vi "Acquire Data.vi"(7 "user event":T2, 8 "error in (no error)":errorcluster, 9 "UI Refs":T1, 10 "Waveforms":waveform(dbl)[](array[waveform]), 11 "H1 Hydraulic":refnum<class "H1 Hydraulic.lvclass">) -> (0 "error out":errorcluster, 3 "H1 Hydraulic out":refnum<class "H1 Hydraulic.lvclass">)   [LabVIEW 2025, in "H1 Plotter.lvlib" / "H1 Hydraulic.lvclass"]
uses:
  H1 Hydraulic.lvclass
  Users/Public/Documents/Sandia National Labs/TSS Plugin/CEF.lvlibp/Node/UserEventRef.ctl
  Users/Public/Documents/Sandia National Labs/TSS Plugin/Tests/XY Plotter.lvlibp/XY Plotter configuration/Read XY Plotter.vi
  Users/Public/Documents/Sandia National Labs/TSS Plugin/CEF.lvlibp/serializable configuration/CEF_serializable configuration.lvclass
  H1 Hydraulic.lvclass/H1 Hydraulic.ctl
  Users/Public/Documents/Sandia National Labs/TSS Plugin/Tests/XY Plotter.lvlibp/XY  Plotter/XY Plotter.lvclass
  Users/Public/Documents/Sandia National Labs/TSS Plugin/CEF.lvlibp/Node/CEF_Node.lvclass
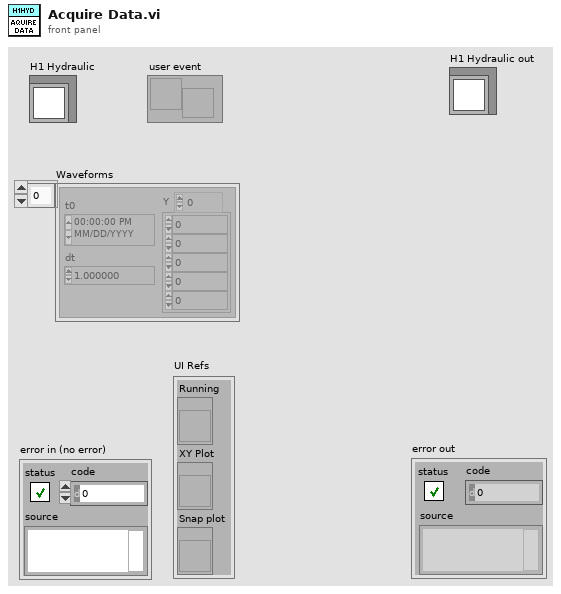
[diagram p1: front panel]
types:
  T1 = cluster{"Running":refnum<vi>, "XY Plot":refnum<vi>, "Snap plot":refnum<vi>}
  T2 = typedef "CEF.lvlibp/CEF_Node.lvclass/UserEventRef.ctl" = refnum<user-event>
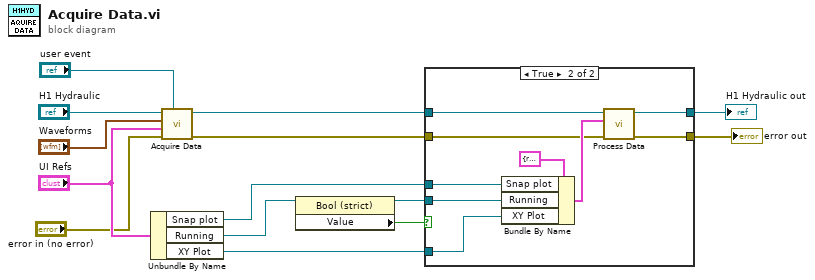
[diagram p0: block diagram]
diagram:
  n1 = Unbundle By Name("UI Refs") -> ("Snap plot"=w8:refnum<vi>, "Running"=w9:refnum<vi>, "XY Plot"=w10:refnum<vi>)
  n2 = call-parent "Acquire Data.vi"("user event"="user event", "error in (no error)"="error in (no error)", "UI Refs"="UI Refs", "Waveforms"="Waveforms", "XY Plotter"="H1 Hydraulic") -> ("error out"=w1:errorcluster, "XY Plotter out"=w6:refnum<class "H1 Hydraulic.lvclass">)  [unwired: 5 in]
  n3 = property class="Bool (strict)"(reference=w9) -> (reference out=w14:refnum<vi>, "Value"=w13:bool)  [unwired: 1 in, 1 out]
  n4 = case shown="True" w13 {
    tunnel: [w16 w25] -> w11
    tunnel: w14 -> [_ w24]
    tunnel: w6 -> [w16 w23]
    tunnel: [w15 w17] -> w12
    tunnel: w10 -> [_ w22]
    tunnel: w8 -> [_ w21]
    tunnel: w1 -> [w15 w18]
    frame False {
    }
    frame True {
      n5 = Bundle By Name(cluster=T1 {"Running"=refnum, "XY Plot"=refnum, "Snap plot"=refnum} ("UI Refs"), "Snap plot"=w21, "Running"=w24, "XY Plot"=w22) -> (w19:T1)
      n6 = call "Process Data.vi"("error in (no error)"=w18, "UI Refs"=w19, "H1 Hydraulic"=w23) -> ("error out"=w17:errorcluster, "H1 Hydraulic out"=w25:refnum<class "H1 Hydraulic.lvclass">)  [unwired: 7 in]
    }
  }
  "error out" <- w12
  "H1 Hydraulic out" <- w11
